vi "fake tool two questions.vi"() -> (0 "error out":errorcluster, 2 "stored":bool, 3 "name":string)   [LabVIEW 2020, in "MCP Server tests.lvlib"]
doc: "Fake tool to test requestState across several rounds (MCP 2026-07-28). It asks two questions in two rounds: first Ask User.vi with the key first (\"What is your name?\", a form with the string property name), then Confirm With User.vi with the key second (\"Store the name?\"). While a question is pending it returns at once without doing anything. name is the name of the first answer, stored is TRUE when the second question was accepted."
uses:
  MCP Server tests.lvlib
  <vilib>/JDP Science/JSONtext/Next JSON Value.vi
  <vilib>/JDP Science/JSONtext/String Subset.vi
  <vilib>/JDP Science/JSONtext/support/Strip Quotes and Unescape.vi
  <vilib>/JDP Science/JSONtext/Parsing/Advance past next JSON Value (inlined COPY).vi
  <vilib>/JDP Science/JSONtext/support/Unescape JSON string.vi
  <vilib>/JDP Science/JSONtext/Parsing/Advance past whitespace.vi
  <vilib>/JDP Science/JSONtext/Parsing/Advance past String.vi
  <vilib>/JDP Science/JSONtext/Parsing/Advance past Number.vi
  <vilib>/JDP Science/JSONtext/Parsing/Advance past Line Ending.vi
  <vilib>/JDP Science/JSONtext/Parsing/Parse Full Path or Item Name.vi
  <vilib>/JDP Science/JSONtext/Parsing/Advance past Array.vi
  <vilib>/JDP Science/JSONtext/Parsing/Advance past Object.vi
  <vilib>/JDP Science/JSONtext/support/Error Cluster From Code.vi
  <vilib>/JDP Science/JSONtext/Offset/Find Item Locations by Path.vi
  <vilib>/JDP Science/JSONtext/Parsing/Advance past next JSON Value.vi
  src/MCP Server/MCP Server.lvlib
  <vilib>/JDP Science/JSONtext/JSONtext.lvlib
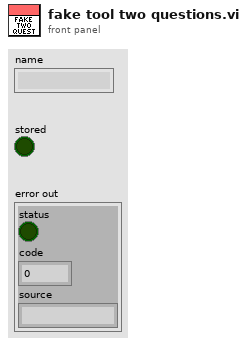
[diagram p1: front panel]
types:
  T1 = enum16{"accept", "decline", "cancel", "pending", "not supported"}
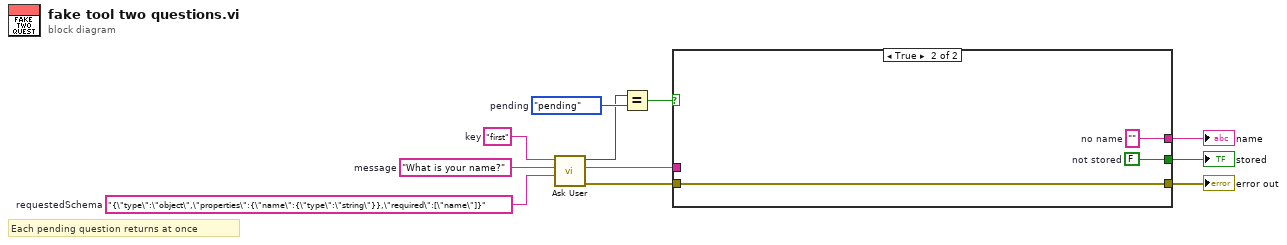
[diagram p0: block diagram]
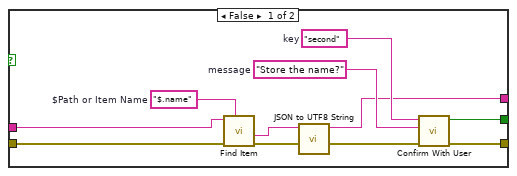
[diagram p2: hidden frame]
diagram:
  w7 = T1."pending"  # pending
  w3 = "{\"type\":\"object\",\"properties\":{\"name\":{\"type\":\"string\"}},\"required\":[\"name\"]}"  # requestedSchema
  w2 = "What is your name?"  # message
  w1 = "first"  # key
  # "Each pending question returns at once"
  n1 = call "Ask User.vi"("requestedSchema"=w3, "message"=w2, "key"=w1) -> ("error out"=w6:errorcluster, "content"=w5:string, "action"=w4:T1)  [unwired: 6 in]
  n2 = Equal?(x=w4, y=w7) -> (x = y?=w8:bool)
  n3 = case shown="True" w8 {
    tunnel: [w17 w24] -> w9
    tunnel: [w21 w25] -> w10
    tunnel: w5 -> [w12 _]
    tunnel: w6 -> [w13 w23]
    tunnel: [w22 w23] -> w11
    frame False {
      w20 = "Store the name?"  # message
      w19 = "second"  # key
      w14 = "$.name"  # $Path or Item Name
      n4 = call <vilib>:"Find Item.vi"("$Path or Item Name"=w14, "error in (no error)"=w13, "JSON"=w12) -> ("error out"=w15:errorcluster, "<JSON>"=w16:string)  [unwired: 5 in, 2 out]
      n5 = call <vilib>:"JSON to UTF8 String.vi"("error in (no error)"=w15, "JSON"=w16) -> ("error out"=w18:errorcluster, "<UTF8>String"=w17:string)  [unwired: 8 in]
      n6 = call "Confirm With User.vi"("error in"=w18, "message"=w20, "key"=w19) -> ("error out"=w22:errorcluster, "confirmed?"=w21:bool)  [unwired: 5 in, 2 out]
    }
    frame True {
      w25 = FALSE  # not stored
      w24 = ""  # no name
    }
  }
  "name" <- w9
  "stored" <- w10
  "error out" <- w11
